vi "P5 Static Events And Timeout.vi"() -> ()   [LabVIEW 2026]
doc: "Round8 probe P5 (UNVERIFIED - prepared 2026-10-22, run when LabVIEW is up): the STATIC-event shape of upstream suite test t88 - a While Loop + Event Structure with two panel Value Change frames (\"Go\" and latched \"Stop\") plus a Timeout frame fed 500 ms through a structure tunnel. No user event, no registration: the interactive-HMI minimal piece. Go Presses and Timeouts are shift registers (Round4/6 idiom: frames read the SR nets directly, every frame assigns every Out tunnel); Stop writes the loop's stop tunnel. Expected on a run that sets Go=true then Stop=true: execState 1, Go Presses >= 1, Timeouts >= 0, Error-free. THE TIMEOUT TUNNEL WIRING IS THE LEAST-CERTAIN PART of this document - if the composer refuses or the VI is broken, inspect how the eventTimeOut terminal is fed before rewriting the frames."
panel:
  out "Timeouts":i32
  out "Go Presses":i32
  in  "Stop":bool
  in  "Go":bool
  in  "Stop":bool
  in  "Go":bool
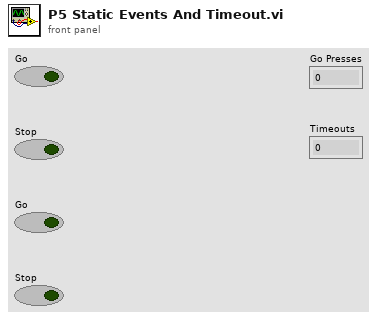
[diagram p1: front panel]
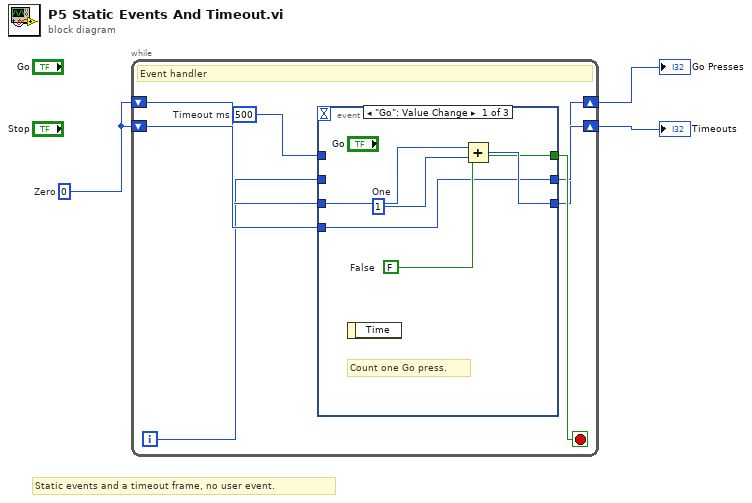
[diagram p0: block diagram]
diagram:
  w1 = 0  # Zero
  # "Static events and a timeout frame, no user event."
  n1 = while {
    shift-right: [w6] -> w2
    shift-left: w1 -> [w5]
    shift-right: [w8] -> w3
    shift-left: w1 -> [w7]
    i -> [w4]
    stop <- w10 stop-if-true
    w9 = 500  # Timeout ms
    # "Event handler"
    n2 = event shown="[0] \"Go\": Value Change" {
      selector: _ -> [_ _ _]
      dyn-events: _ -> [_ _ _]
      timeout: _ -> [_ _ _]
      tunnel: w9 -> [_ _ _]
      tunnel: w4 -> [_ _ _]
      tunnel: [w14 w19 TRUE] -> w10
      tunnel: w5 -> [w11 w16 w21]
      tunnel: w7 -> [w12 w17 w22]
      tunnel: [w12 w20 w22] -> w8
      tunnel: [w15 w16 w21] -> w6
      event "Go": Value Change {
        w14 = FALSE  # False
        w13 = 1  # One
        # "Count one Go press."
        n3 = event-data() -> ()  [unwired: 1 in, 3 out]
        n4 = Add(x=w11, y=w13) -> (x+y=w15:i32)
      }
      event Timeout {
        w19 = FALSE  # False
        w18 = 1  # One
        # "Count one timeout tick."
        n5 = event-data() -> ()  [unwired: 1 in, 3 out]
        n6 = Add(x=w17, y=w18) -> (x+y=w20:i32)
      }
      event "Stop": Value Change {
        # "Latched Stop ends the loop."
        n7 = event-data() -> ()  [unwired: 1 in, 3 out]
      }
    }
  }
  "Go Presses" <- w2
  "Timeouts" <- w3
